vi "libssh2_agent_set_identity_path.vi"(8 "error in (no error)":errorcluster, 10 "path":path, 11 "agent":T1) -> (0 "error out":errorcluster)   [LabVIEW 2017, in "libssh2.lvlib"]
doc: "Set the path to a custom identity socket instead of the default <B>SSH_AUTH_SOCK</B> environment variable."
uses:
  libssh2.lvlib
  Agent Refnum.ctl
  Acquire Session.vi
  Release Session.vi
  Not An Agent.vi
  <vilib>/Utility/error.llb/Error Cluster From Error Code.vi
  Global Settings.vi
  Read Agent Refnum.vi
  Read Session Refnum.vi
  <vilib>/Utility/semaphor.llb/Acquire Semaphore.vi
  <vilib>/Utility/semaphor.llb/Release Semaphore.vi
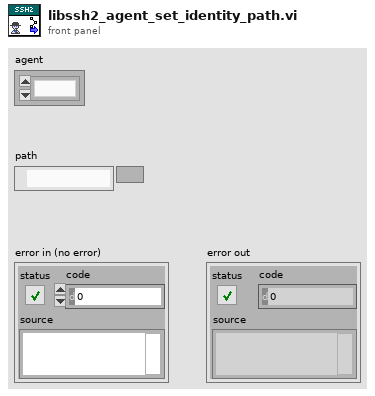
[diagram p1: front panel]
types:
  T1 = typedef "libssh2.lvlib/Agent Refnum.ctl" = refnum<k1>
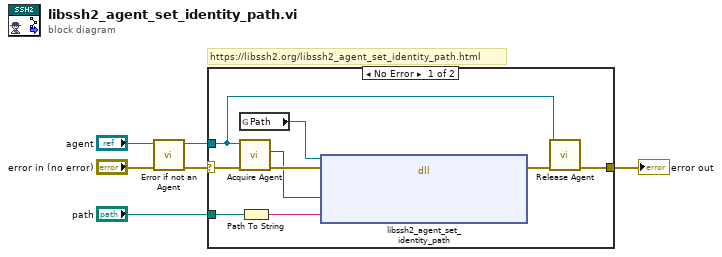
[diagram p0: block diagram]
diagram:
  # "https://libssh2.org/libssh2_agent_set_identity_path.html"
  n1 = call "Error if not an Agent.vi"("error in (no error)"="error in (no error)", "agent"="agent") -> ("error out"=w3:errorcluster, "agent out"=w1:T1)  [unwired: 8 in]
  n2 = case shown="No Error" w3 {
    selector: w3 -> [w15 w16]
    tunnel: [w8 w16] -> w6
    tunnel: w1 -> [w7 _]
    tunnel: "path" -> [w14 _]
    frame No Error {
      n3 = global read "Global Settings.vi" "Path"() -> (w13:path)
      n4 = call "Acquire Agent.vi"("error in (no error)"=w15, "agent"=w7) -> ("error out"=w12:errorcluster, "LIBSSH2_AGENT*"=w11:u64)  [unwired: 8 in]
      n5 = Path To String(path=w14) -> (string=w10:string)
      n6 = dll-call lib="?" fn="libssh2_agent_set_identity_path"(path in=w13, error in=w12, "agent"=w11, "path"=w10) -> (error out=w9:errorcluster)  [unwired: 4 in, 1 out]
      n7 = call "Release Agent.vi"("error in (no error)"=w9, "agent"=w7) -> ("error out"=w8:errorcluster)  [unwired: 9 in]
    }
    frame Error {
    }
  }
  "error out" <- w6
